vi "Map Tags to Channels.vi"(7 "instance id":string, 8 "error in (no error)":errorcluster, 9 "String Array":string[][](array[string]), 10 "Lines":T1[](array[typedef]), 11 "engine configuration in":refnum<class "engine configuration.lvclass">) -> (0 "error out":errorcluster, 3 "engine configuration out":refnum<class "engine configuration.lvclass">)   [LabVIEW 2015, in "PID Module editor node.lvclass"]
uses:
  PID Module editor node.lvclass
  module/configuration/Line.ctl
  <vilib>/NI/Tag Bus Module Framework/channel/TBM channel.lvclass
  <vilib>/NI/Module Execution Interface/Engine Configuration/engine configuration.lvclass
  <vilib>/NI/Tag Bus/tag/tag descriptor.lvclass/tag descriptor.ctl
  <vilib>/NI/Tag Bus/tag/tag descriptor.lvclass
  module/configuration/PID Module configuration.lvclass
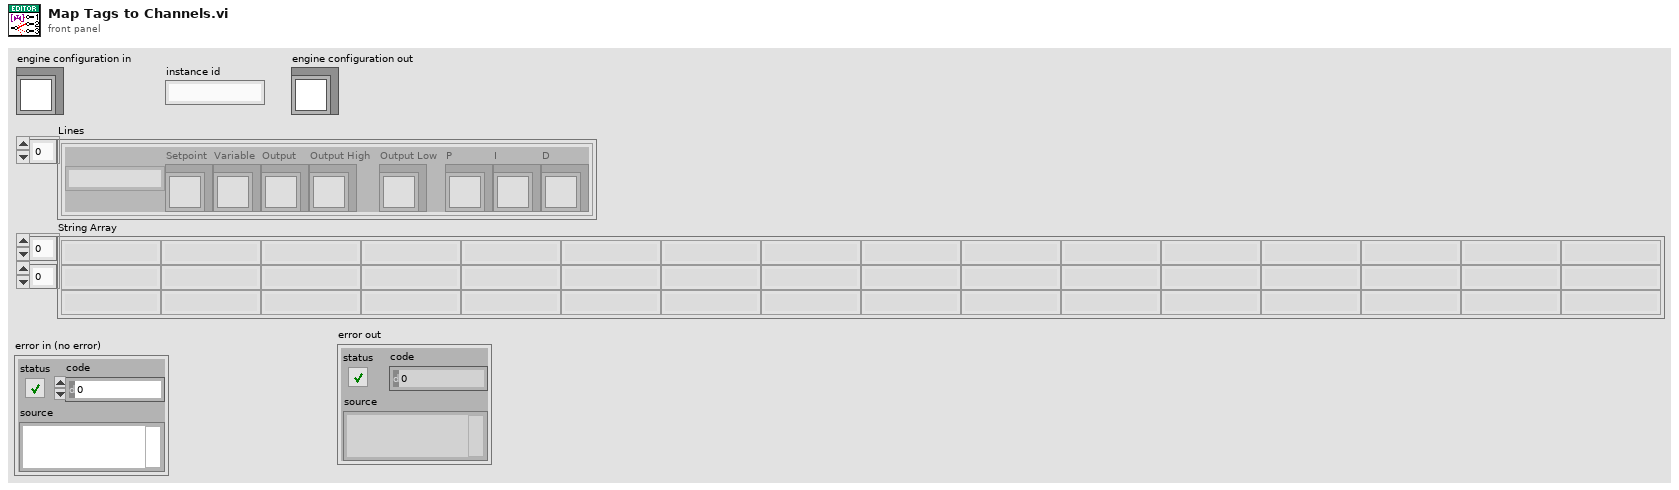
[diagram p1: front panel]
types:
  T1 = typedef "PID Module configuration.lvclass/Line.ctl" = cluster{"PID ID":string, "Setpoint":refnum<class "TBM channel.lvclass">, "Variable":refnum<class "TBM channel.lvclass">, "Output":refnum<class "TBM channel.lvclass">, "Output High":refnum<class "TBM channel.lvclass">, "Output Low":refnum<class "TBM channel.lvclass">, "P":refnum<class "TBM channel.lvclass">, "I":refnum<class "TBM channel.lvclass">, "D":refnum<class "TBM channel.lvclass">}
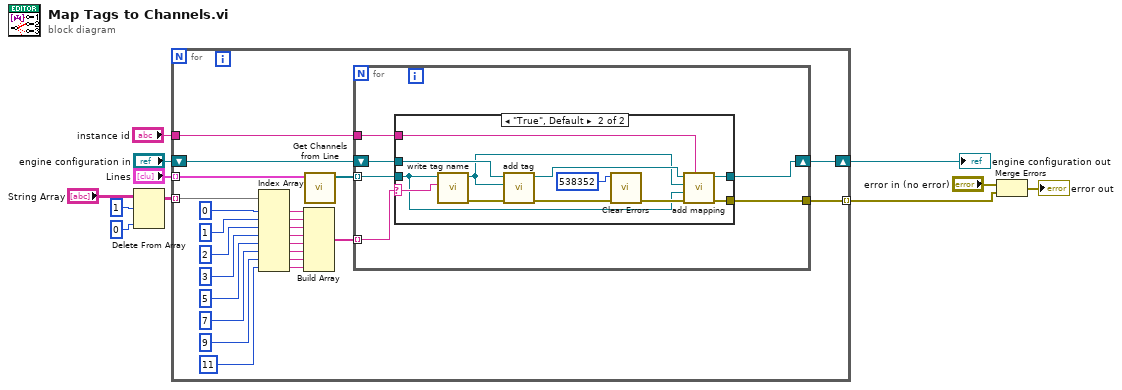
[diagram p0: block diagram]
diagram:
  n1 = Delete From Array(array="String Array", length=1, index (col)=0 ("disabled index (col)")) -> (array with subset deleted=w1:string[][])  [unwired: 1 in, 1 out]
  n2 = for {
    tunnel: "Lines" -> [w31] mode=indexing
    tunnel: w1 -> [w29] mode=indexing
    shift-right: [w35] -> w8
    shift-left: "engine configuration in" -> [w32]
    tunnel: "instance id" -> [w34]
    tunnel: [w33] -> w10 mode=indexing
    n3 = Index Array(array=w29, index #1=0 ("index"), index #2=1 ("index"), index #3=2 ("index"), index #4=3 ("index"), index #5=5 ("index"), index #6=7 ("index"), index #7=9 ("index"), index #8=11 ("index")) -> (element #1=w21:string, element #2=w20:string, element #3=w19:string, element #4=w16:string, element #5=w15:string, element #6=w14:string, element #7=w13:string, element #8=w12:string)
    n4 = Build Array(w21, w20, w19, w16, w15, w14, w13, w12) -> (w18:string[])
    n5 = call "Get Channels from Line.vi"("Line"=w31) -> ("Channels"=w30:refnum<class "TBM channel.lvclass">[])  [unwired: 10 in]
    n6 = for {
      tunnel: w34 -> [w40]
      tunnel: [w39] -> w33
      tunnel: w30 -> [w37] mode=indexing
      tunnel: w18 -> [w36] mode=indexing
      shift-right: [w41] -> w35
      shift-left: w32 -> [w38]
      n7 = case shown="\"True\", Default" w36 {
        selector: w36 -> [_ w45]
        tunnel: [w42 w54] -> w41
        tunnel: w40 -> [_ w53]
        tunnel: [_ w52] -> w39
        tunnel: w38 -> [w42 w51]
        tunnel: w37 -> [_ w43]
        frame "" {
        }
        frame "True", Default {
          n8 = call <vilib>:"write tag name.vi"("name"=w45, "system tag in"=w43) -> ("error out"=w49:errorcluster, "system tag out"=w44:refnum<class "TBM channel.lvclass">)  [unwired: 8 in]
          n9 = call-dynamic "add tag.vi"("error in"=w49, "tag descriptor"=w44, "engine configuration in"=w51) -> ("error out"=w48:errorcluster, "engine configuration out"=w50:refnum<class "engine configuration.lvclass">)  [unwired: 7 in]
          n10 = call <vilib>:"Clear Errors.vi"("error in (no error)"=w48, "specific error code to clear (0: all)"=538352) -> ("error out"=w47:errorcluster)  [unwired: 4 in, 1 out]
          n11 = call-dynamic "add mapping.vi"("owner ID"=w53, "error in"=w47, "channel"=w43, "tag descriptor"=w44, "engine configuration"=w50) -> ("error out"=w52:errorcluster, "engine configuration out"=w54:refnum<class "engine configuration.lvclass">)  [unwired: 5 in]
        }
      }
    }
  }
  "engine configuration out" <- w8
  n12 = Merge Errors("error in (no error)", w10) -> (→"error out":errorcluster)
